vi "Get Analog Cluster.vi"() -> (2 "Analog Output List":T1[](array[typedef]), 3 "Analog Input List":T1[](array[typedef]))   [LabVIEW 2021]
uses:
  DAQNav/Analog Cluster.ctl
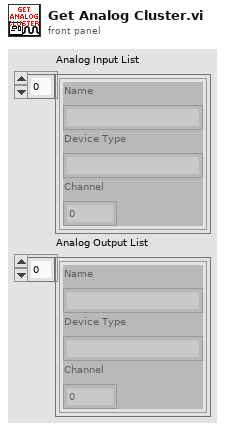
[diagram p1: front panel]
types:
  T1 = typedef "Analog Cluster.ctl" = cluster{"Name":string, "Device Type":string, "Channel":i32}
  T2 = typedef "Device Settings.ctl" = cluster{"Session":string, "Key and Value":string[][]}
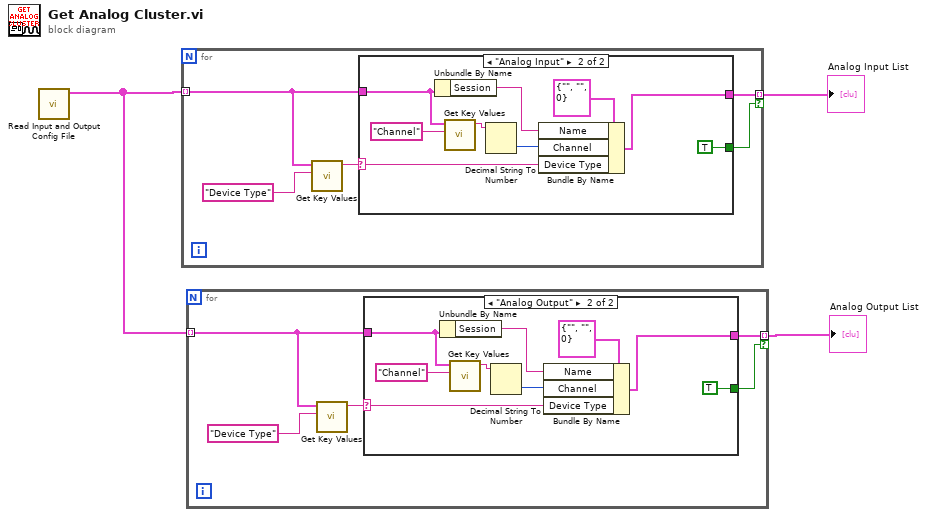
[diagram p0: block diagram]
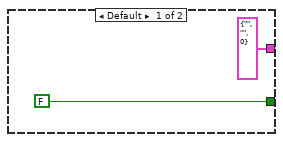
[diagram p2: hidden frame]
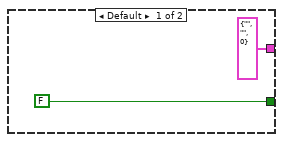
[diagram p3: hidden frame]
diagram:
  n1 = call "Read Input and Output Config File.vi"() -> ("Input and Output Settings"=w1:T2[])  [unwired: 10 in, 1 out]
  n2 = for {
    tunnel: w1 -> [w6] mode=indexing
    tunnel: [w5] -> w3 mode=indexing if=w4
    n3 = call "Get Key Values.vi"("Search Key"="Device Type" ("key"), "Configure Cluster"=w6) -> ("value"=w7:string)  [unwired: 8 in, 1 out]
    n4 = case shown="\"Analog Input\"" w7 {
      selector: w7 -> [_ w16]
      tunnel: w6 -> [_ w15]
      tunnel: [T1 {"Name"="", "Device Type"="", "Channel"=0} w11] -> w5
      tunnel: [FALSE TRUE] -> w4
      frame Default {
      }
      frame "Analog Input" {
        n5 = Unbundle By Name(w15) -> ("Session"=w14:string)
        n6 = call "Get Key Values.vi"("Search Key"="Channel" ("key"), "Configure Cluster"=w15) -> ("value"=w13:string)  [unwired: 8 in, 1 out]
        n7 = Decimal String To Number(string=w13) -> (number=w12:i32)  [unwired: 2 in, 1 out]
        n8 = Bundle By Name(cluster=T1 {"Name"="", "Device Type"="", "Channel"=0}, "Name"=w14, "Channel"=w12, "Device Type"=w16) -> (w11:T1)
      }
    }
  }
  "Analog Input List" <- w3
  n9 = for {
    tunnel: w1 -> [w22] mode=indexing
    tunnel: [w21] -> w2 mode=indexing if=w20
    n10 = call "Get Key Values.vi"("Search Key"="Device Type" ("key"), "Configure Cluster"=w22) -> ("value"=w23:string)  [unwired: 8 in, 1 out]
    n11 = case shown="\"Analog Output\"" w23 {
      selector: w23 -> [_ w32]
      tunnel: w22 -> [_ w31]
      tunnel: [T1 {"Name"="", "Device Type"="", "Channel"=0} w27] -> w21
      tunnel: [FALSE TRUE] -> w20
      frame Default {
      }
      frame "Analog Output" {
        n12 = Unbundle By Name(w31) -> ("Session"=w30:string)
        n13 = call "Get Key Values.vi"("Search Key"="Channel" ("key"), "Configure Cluster"=w31) -> ("value"=w29:string)  [unwired: 8 in, 1 out]
        n14 = Decimal String To Number(string=w29) -> (number=w28:i32)  [unwired: 2 in, 1 out]
        n15 = Bundle By Name(cluster=T1 {"Name"="", "Device Type"="", "Channel"=0}, "Name"=w30, "Channel"=w28, "Device Type"=w32) -> (w27:T1)
      }
    }
  }
  "Analog Output List" <- w2
